vi "Analysis Produces Correct number of Type Definitions .vi"(11 "Test Case In":refnum<class "Python Code Analysis.lvclass">) -> (0 "error out":errorcluster, 3 "Test Case Out":refnum<class "Python Code Analysis.lvclass">)   [LabVIEW 2026, in "Python Code Analysis.lvclass"]
doc: "This tests that the analysis of the dummy python module produces the correct amount of type definitions."
uses:
  Python Code Analysis.lvclass
  C:/Program Files/National Instruments/LabVIEW 2026/vi.lib/Astemes/LUnit/Test Case.lvclass
  <vilib>/Astemes/LUnit/Test Case.lvclass/Test Case.ctl
  <vilib>/Astemes/LUnit/Core/LUnit Test Case/Private/Append Fail Result.vi
  <vilib>/Astemes/LUnit/Core/LUnit Test Case/Private/Append Pass Result.vi
  <vilib>/Astemes/LUnit/Core/LUnit Test Case/Private/Run In UI.vi
  <vilib>/Utility/error.llb/Clear Errors.vi
  Python Code Analysis.lvclass/Python Code Analysis.ctl
  <vilib>/Astemes/LUnit/Test Case.lvclass
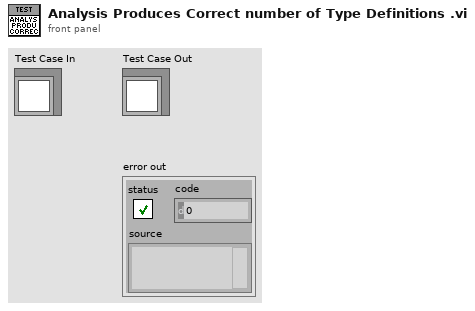
[diagram p1: front panel]
types:
  T1 = typedef "Analysis Output--cluster.ctl" = cluster{"type_definitions":T2[], "functions":T4[]}
  T2 = typedef "Type Definition--cluster.ctl" = cluster{"name":string, "fields":T3[]}
  T3 = typedef "Parameter--cluster.ctl" = cluster{"name":string, "data_type":string, "container":string, "dimensions":i32, "type_definition":string}
  T4 = typedef "Function--cluster.ctl" = cluster{"name":string, "docstring":string, "input_parameters":T3[], "output_parameters":T3[]}
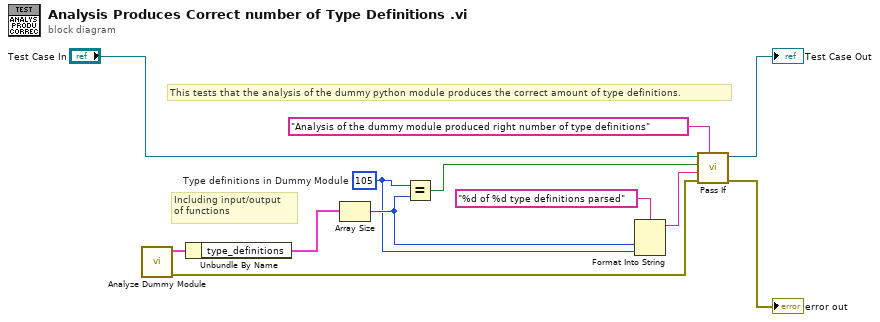
[diagram p0: block diagram]
diagram:
  w3 = 105  # Type definitions in Dummy Module
  # "Including input/output\nof functions"
  # "This tests that the analysis of the dummy python module produces the correct amount of type definitions."
  n1 = call "Analyze Dummy Module.vi"() -> ("error out"=w11:errorcluster, "Analysis Output"=w7:T1)  [unwired: 10 in]
  n2 = Unbundle By Name(w7) -> ("type_definitions"=w8:T2[])
  n3 = Array Size(array=w8) -> (size(s)=w4:i32)
  n4 = Equal?(x=w3, y=w4) -> (x = y?=w6:bool)
  n5 = Format Into String(format string="%d of %d type definitions parsed", w4, w3) -> (resulting string=w2:string)  [unwired: 2 in, 1 out]
  n6 = call <vilib>:"Pass If.vi"("Description"="Analysis of the dummy module produced right number of type definitions", "error in (no error)"=w11, "Message"=w2, "Pass?"=w6, "LUnit Test Case In"="Test Case In") -> ("error out"=→"error out":errorcluster, "LUnit Test Case Out"=→"Test Case Out":refnum<class "Python Code Analysis.lvclass">)  [unwired: 5 in]
